vi "fetch TXP Value.vi"(8 "error in (no error)":errorcluster, 11 "Keysight 9020A in":refnum<class "Keysight 9020A.lvclass">) -> (0 "error out":errorcluster, 2 "TXP Value":dbl[](array[numeric]), 3 "Keysight 9020A out":refnum<class "Keysight 9020A.lvclass">)   [LabVIEW 2023, in "Spectrum Analyzer.lvlib" / "Keysight 9020A.lvclass"]
uses:
  Keysight 9020A.lvclass
  Keysight 9020A.lvclass/Keysight 9020A.ctl
  Spectrum Analyzer.lvlib
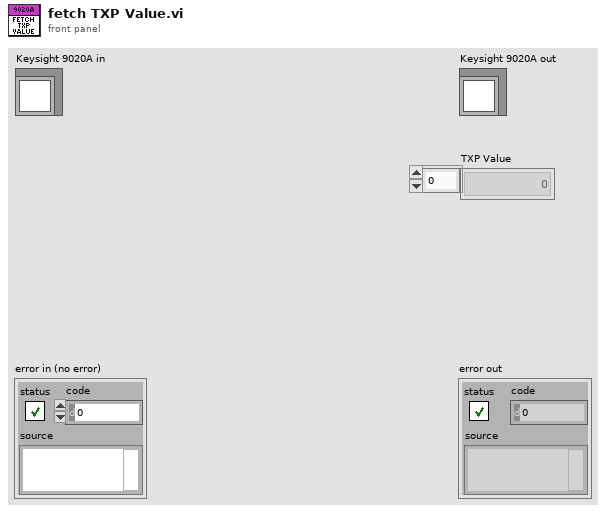
[diagram p1: front panel]
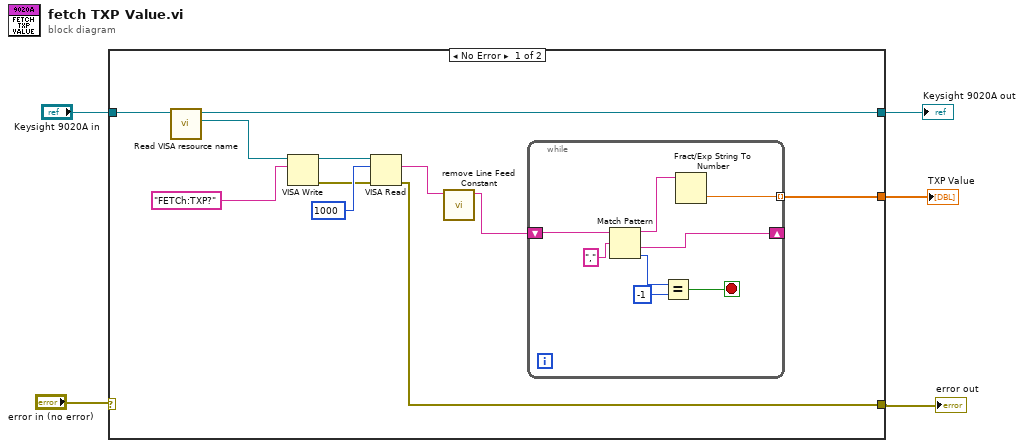
[diagram p0: block diagram]
diagram:
  n1 = case shown="No Error" "error in (no error)" {
    selector: "error in (no error)" -> [_ w25]
    tunnel: "Keysight 9020A in" -> [w14 w26]
    tunnel: [w16 w26] -> w4
    tunnel: [w9 w25] -> w1
    tunnel: [w6 _] -> w3
    frame No Error {
      n2 = call "Read VISA resource name.vi"("Keysight 9020A in"=w14) -> ("VISA resource name"=w15:refnum<visa-resource-name>, "Keysight 9020A out"=w16:refnum<class "Keysight 9020A.lvclass">)  [unwired: 8 in, 1 out]
      n3 = VISA Write(VISA resource name=w15, write buffer="FETCh:TXP?") -> (VISA resource name out=w12:refnum<visa-resource-name>, error out=w11:errorcluster)  [unwired: 1 in, 1 out]
      n4 = VISA Read(VISA resource name=w12, byte count=u32 1000, error in (no error)=w11) -> (read buffer=w10:string, error out=w9:errorcluster)  [unwired: 2 out]
      n5 = call "remove Line Feed Constant.vi"("Input String"=w10) -> ("Line Feed Removed String"=w7:string)  [unwired: 10 in]
      n6 = while {
        shift-right: [w22] -> _
        shift-left: w7 -> [w24]
        tunnel: [w20] -> w6 mode=indexing
        stop <- w17 stop-if-true
        n7 = Match Pattern(string=w24, regular expression=",") -> (before substring=w21:string, after substring=w22:string, offset past match=w19:i32)  [unwired: 1 in, 1 out]
        n8 = Equal?(x=w19, y=-1) -> (x = y?=w17:bool)
        n9 = Fract/Exp String To Number(string=w21) -> (number=w20:dbl)  [unwired: 3 in, 1 out]
      }
    }
    frame Error {
    }
  }
  "error out" <- w1
  "Keysight 9020A out" <- w4
  "TXP Value" <- w3
